vi "Release Valid Builder Reference.vi"(8 "error in (no error)":errorcluster, 11 "reference":T1) -> (0 "error out":errorcluster)   [LabVIEW 2026, in "ToastNotification.lvlib" / "ToastBuilder.lvclass"]
doc: "Release a valid builder handle even with an incoming error. Ignore null or already closed handles. Merge the incoming error before the cleanup error. Does not call Dispose or unregister events; closing a shared handle invalidates its aliases."
uses:
  ToastBuilder.lvclass
  Builder Reference.ctl
  C:/Users/loicw/Documents/LabVIEW/ToastNotifications/Sources/bins/Microsoft.Toolkit.Uwp.Notifications.dll
  bins/Microsoft.Toolkit.Uwp.Notifications.dll
  ToastBuilder.lvclass/ToastBuilder.ctl
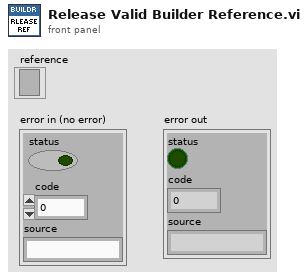
[diagram p1: front panel]
types:
  T1 = typedef "ToastNotification.lvlib/ToastBuilder.lvclass/Builder Reference.ctl" = refnum<k24>
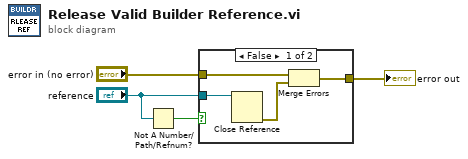
[diagram p0: block diagram]
diagram:
  n1 = Not A Number/Path/Refnum?(number/path/refnum="reference") -> (NaN/Path/Refnum?=w3:bool)
  n2 = case shown="False" w3 {
    tunnel: "reference" -> [w5 _]
    tunnel: "error in (no error)" -> [w6 w9]
    tunnel: [w8 w9] -> w4
    frame False {
      n3 = Close Reference(reference=w5) -> (error out=w7:errorcluster)  [unwired: 1 in]
      n4 = Merge Errors(w6, w7) -> (w8:errorcluster)
    }
    frame True {
    }
  }
  "error out" <- w4
